vi "CreateFolder.vi"(1 "folder name":string, 3 "Path in":path) -> (0 "path out":path)   [LabVIEW 2025]
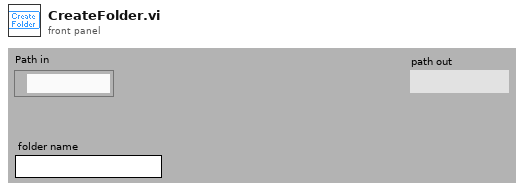
[diagram p1: front panel]
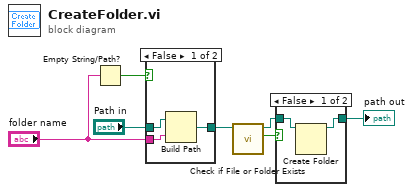
[diagram p0: block diagram]
diagram:
  n1 = Empty String/Path?(string/path="folder name") -> (empty?=w1:bool)
  n2 = case shown="False" w1 {
    tunnel: "Path in" -> [w10 w11]
    tunnel: [w9 w11] -> w6
    tunnel: "folder name" -> [w8 _]
    frame False {
      n3 = Build Path(base path=w10, name or relative path=w8) -> (appended path=w9:path)
    }
    frame True {
    }
  }
  n4 = call <vilib>:"Check if File or Folder Exists.vi"("path"=w6) -> ("file or folder exists?"=w5:bool, "dup path"=w4:path)  [unwired: 1 in, 8 out]
  n5 = case shown="False" w5 {
    tunnel: w4 -> [w13 w14]
    tunnel: [w12 w14] -> w3
    frame False {
      n6 = Create Folder(path (use dialog)=w13) -> (created path=w12:path)  [unwired: 1 in, 3 out]
    }
    frame True {
    }
  }
  "path out" <- w3
